vi "lab-pid.vi"() -> ()   [LabVIEW 2022 SP3]
uses:
  <vilib>/Instr/_visa.llb/VISA Configure Serial Port (Instr).vi
  <vilib>/addons/control/pid/pid.llb/PID (DBL).vi
  <vilib>/addons/control/pid/NI_PID_pid.lvlib
panel:
  out "pid out":dbl format="%.2f"
  in  "PID gains":T1={"proportional gain (Kc)"=1.0, "integral time (Ti, min)"=0.01, "derivative time (Td, min)"=0.0} {"derivative time (Td, min)" format="%.3f"; "integral time (Ti, min)" format="%.3f"; "proportional gain (Kc)" format="%.3f"}
  out "pwm":dbl
  out "elev":dbl
  in  "stop":bool
  in  "target":dbl
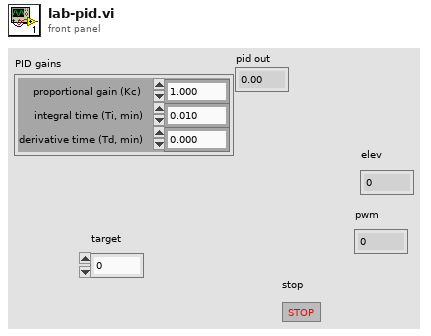
[diagram p1: front panel]
types:
  T1 = cluster{"proportional gain (Kc)":dbl, "integral time (Ti, min)":dbl, "derivative time (Td, min)":dbl}
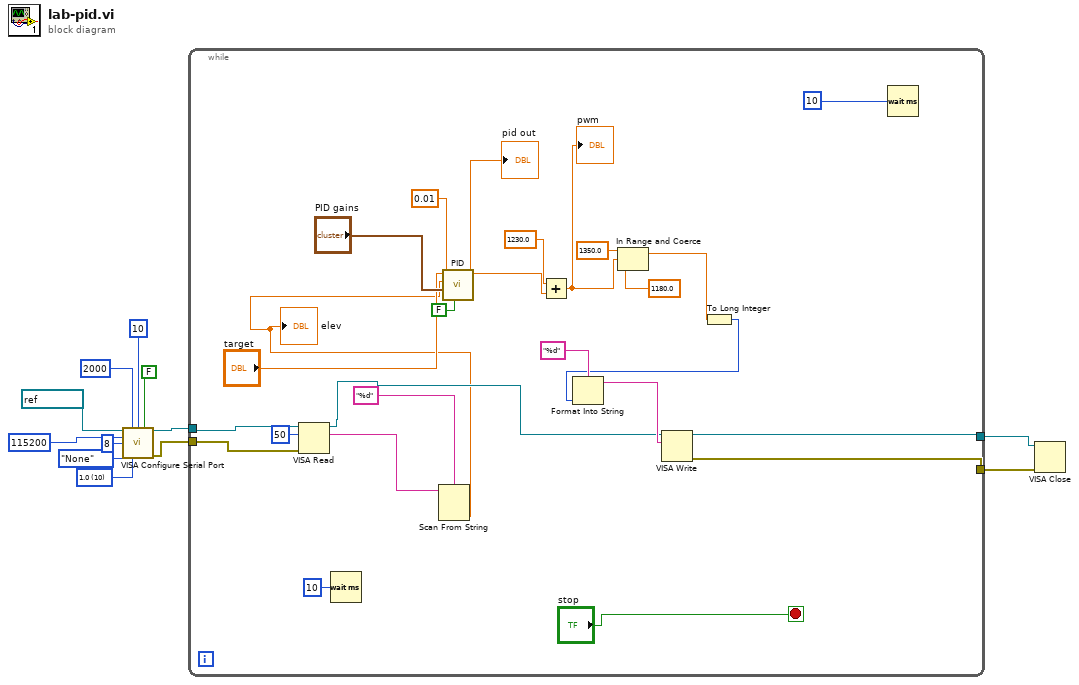
[diagram p0: block diagram]
diagram:
  w9 = u16 10 items=["1.0"=10, "1.5"=15, "2.0"=20] ("stop bits (10: 1 bit)")
  n1 = call-poly "VISA Configure Serial Port"("VISA resource name"=refnum<visa-resource-name> "COM4", "timeout (10sec)"=u32 2000, "termination char\n(0xA = '\\n' = LF)"=u8 10 ("termination char\n(0xA = '\\n' = LF)"), "Enable Termination\nChar (T)"=FALSE ("Enable Termination\nChar (T)"), "baud rate (9600)"=u32 115200, "data bits (8)"=u16 8, "parity (0:none)"=enum16{"None", "Odd", "Even", "Mark", "Space"}."None", "stop bits (10: 1 bit)"=w9) -> ("VISA resource name out"=w4:refnum<visa-resource-name>, "error out"=w3:errorcluster)  [unwired: 6 in]
  n2 = while {
    tunnel: w4 -> [w21]
    tunnel: w3 -> [w34]
    tunnel: [w16] -> w2
    tunnel: [w15] -> w1
    stop <- "stop" stop-if-true
    n3 = VISA Read(VISA resource name=w21, byte count=u32 50, error in (no error)=w34) -> (VISA resource name out=w20:refnum<visa-resource-name>, read buffer=w35:string)  [unwired: 2 out]
    n4 = Wait (ms)(milliseconds to wait=u32 10) -> ()  [unwired: 1 out]
    n5 = Scan From String(format string="%d", input string=w35) -> (output 1=w13:dbl)  [unwired: 3 in, 3 out]
    "elev" <- w13
    n6 = call-poly <vilib>:"PID.vi"("reinitialize? (F)"=FALSE, "dt (s)"=0.01, "PID gains"="PID gains", "process variable"=w13, "setpoint"="target") -> ("output"=w29:dbl)  [unwired: 5 in, 1 out]
    "pid out" <- w29
    n7 = Add(x=1230.0, y=w29) -> (x+y=w25:dbl)
    "pwm" <- w25
    n8 = In Range and Coerce(upper limit=1350.0, x=w25, lower limit=1180.0) -> (coerced(x)=w24:dbl)  [unwired: 1 out]
    n9 = To Long Integer(number=w24) -> (32bit integer=w18:i32)
    n10 = Format Into String(format string="%d", w18) -> (resulting string=w22:string)  [unwired: 2 in, 1 out]
    n11 = VISA Write(VISA resource name=w20, write buffer=w22) -> (VISA resource name out=w16:refnum<visa-resource-name>, error out=w15:errorcluster)  [unwired: 1 in, 1 out]
    n12 = Wait (ms)(milliseconds to wait=u32 10) -> ()  [unwired: 1 out]
  }
  n13 = VISA Close(VISA resource name=w2, error in (no error)=w1) -> ()  [unwired: 1 out]
